vi "NSA Call Process.vi"(8 "error in (no error)":errorcluster caption="에러 입력(에러 없음)", 10 "NSA Call Process Param":T1, 11 "Instrument Manager 입력":refnum<class "Instrument Manager.lvclass">) -> (0 "error out":errorcluster caption="에러 출력", 3 "Instrument Manager 출력":refnum<class "Instrument Manager.lvclass">)   [LabVIEW 2023, in "Instrument Manager.lvclass"]
uses:
  Instrument Manager.lvclass
  Param Definition/NSA Call Process Param.ctl
  Module/ANRITSU Call Box/Type Definition/NR Modulation Type.ctl
  Instrument Manager.lvclass/Instrument Manager.ctl
  97ae3937-7c23-4982-aa73-e3704093bdd1.vi
  Module/ANRITSU Call Box/ANRITSU Call Box.lvlib
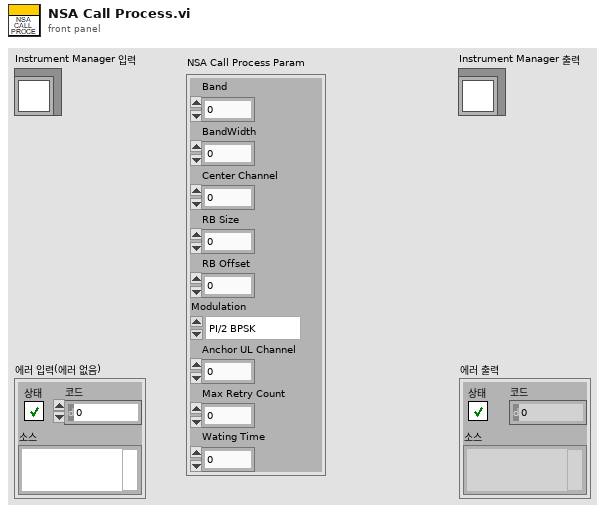
[diagram p1: front panel]
types:
  T1 = typedef "NSA Call Process Param.ctl" = cluster{"Band":u32, "BandWidth":u32, "Center Channel":u32, "RB Size":i32, "RB Offset":i32, "Modulation":T2, "Anchor UL Channel":i32, "Max Retry Count":i32, "Wating Time":i32}
  T2 = typedef "ANRITSU Call Box.lvlib/NR Modulation Type.ctl" = enum16{"PI/2 BPSK", "QPSK", "16QAM", "64QAM", "256QAM"}
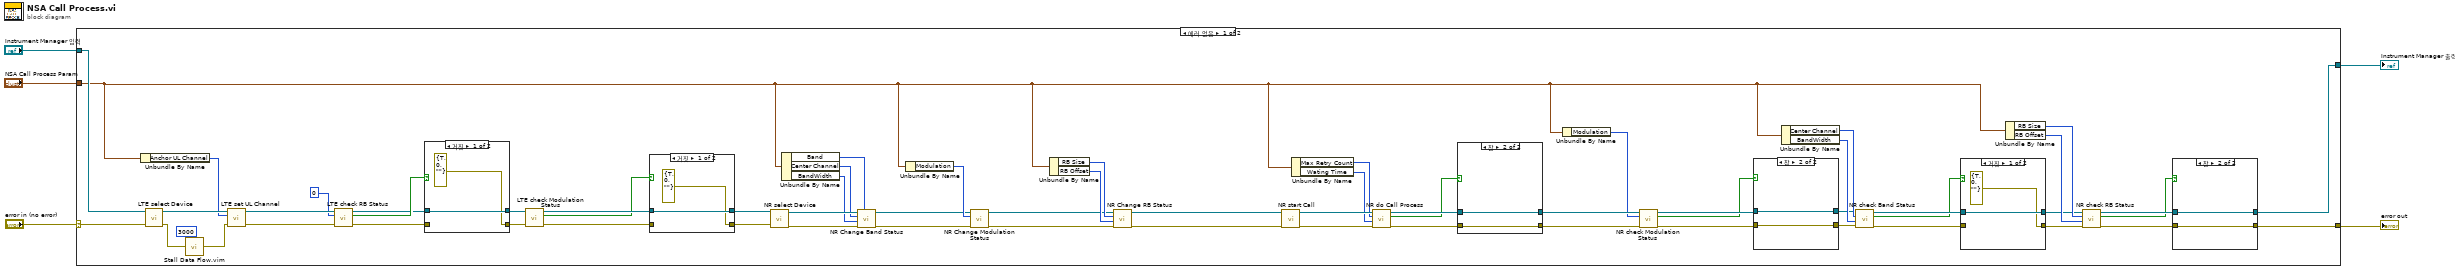
[diagram p0: block diagram]
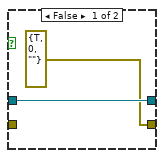
[diagram p2: hidden frame]
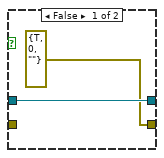
[diagram p4: hidden frame]
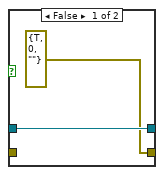
[diagram p5: hidden frame]
diagram:
  n1 = case shown="에러 없음" "error in (no error)" {
    selector: "error in (no error)" -> [w56 w95]
    tunnel: [w12 w95] -> w4
    tunnel: [w9 w94] -> w2
    tunnel: "Instrument Manager 입력" -> [w55 w94]
    tunnel: "NSA Call Process Param" -> [w21 _]
    frame No Error {
      n2 = Unbundle By Name(w21) -> ("Anchor UL Channel"=w58:i32)
      n3 = call "LTE select Device.vi"("error in (no error)"=w56, "Instrument Manager 입력"=w55) -> ("error out"=w8:errorcluster, "Instrument Manager 출력"=w61:refnum<class "Instrument Manager.lvclass">)  [unwired: 8 in]
      n4 = call "Stall Data Flow.vim"("value in"=w8, "milliseconds to wait"=u32 3000) -> ("value out"=w7:errorcluster)  [unwired: 1 out]
      n5 = call "LTE set UL Channel.vi"("error in (no error)"=w7, "UL Channel"=w58, "Instrument Manager 입력"=w61) -> ("error out"=w59:errorcluster, "Instrument Manager 출력"=w60:refnum<class "Instrument Manager.lvclass">)  [unwired: 7 in]
      n6 = call "LTE check RB Status.vi"("error in (no error)"=w59, "RB Offset"=0, "Instrument Manager 입력"=w60) -> ("error out"=w62:errorcluster, "불리언"=w64:bool, "Instrument Manager 출력"=w63:refnum<class "Instrument Manager.lvclass">)  [unwired: 6 in]
      n7 = case shown="거짓" w64 {
        tunnel: w63 -> [w91 w93]
        tunnel: [w91 w93] -> w66
        tunnel: [errorcluster {"status"=TRUE, "code"=0, "source"=""} ("error out") w92] -> w65
        tunnel: w62 -> [_ w92]
        frame False {
        }
        frame True {
        }
      }
      n8 = call "LTE check Modulation Status.vi"("error in (no error)"=w65, "Instrument Manager 입력"=w66) -> ("error out"=w68:errorcluster, "불리언"=w67:bool, "Instrument Manager 출력"=w69:refnum<class "Instrument Manager.lvclass">)  [unwired: 7 in]
      n9 = case shown="거짓" w67 {
        tunnel: w69 -> [w87 w89]
        tunnel: [w87 w89] -> w25
        tunnel: [errorcluster {"status"=TRUE, "code"=0, "source"=""} ("error out") w88] -> w26
        tunnel: w68 -> [_ w88]
        frame False {
        }
        frame True {
        }
      }
      n10 = call "NR select Device.vi"("error in (no error)"=w26, "Instrument Manager 입력"=w25) -> ("error out"=w53:errorcluster, "Instrument Manager 출력"=w54:refnum<class "Instrument Manager.lvclass">)  [unwired: 8 in]
      n11 = Unbundle By Name(w21) -> ("Band"=w31:u32, "Center Channel"=w30:u32, "BandWidth"=w29:u32)
      n12 = call "NR Change Band Status.vi"("Operation Band"=w31, "error in (no error)"=w53, "BW (MHz)"=w29, "Center Channel Number"=w30, "Instrument Manager 입력"=w54) -> ("error out"=w28:errorcluster, "Instrument Manager 출력"=w27:refnum<class "Instrument Manager.lvclass">)  [unwired: 5 in]
      n13 = Unbundle By Name(w21) -> ("Modulation"=w32:T2)
      n14 = call "NR Change Modulation Status.vi"("error in (no error)"=w28, "Modulation"=w32, "Instrument Manager 입력"=w27) -> ("error out"=w37:errorcluster, "Instrument Manager 출력"=w38:refnum<class "Instrument Manager.lvclass">)  [unwired: 7 in]
      n15 = Unbundle By Name(w21) -> ("RB Size"=w40:i32, "RB Offset"=w39:i32)
      n16 = call "NR Change RB Status.vi"("error in (no error)"=w37, "RB Offset"=w39, "RB Size"=w40, "Instrument Manager 입력"=w38) -> ("error out"=w49:errorcluster, "Instrument Manager 출력"=w51:refnum<class "Instrument Manager.lvclass">)  [unwired: 6 in]
      n17 = call "NR start Call.vi"("error in (no error)"=w49, "Instrument Manager 입력"=w51) -> ("error out"=w50:errorcluster, "Instrument Manager 출력"=w52:refnum<class "Instrument Manager.lvclass">)  [unwired: 8 in]
      n18 = Unbundle By Name(w21) -> ("Max Retry Count"=w45:i32, "Wating Time"=w44:i32)
      n19 = call "NR do Call Process.vi"("error in (no error)"=w50, "Waiting Time"=w44, "Max Retry Count"=w45, "Instrument Manager 입력"=w52) -> ("error out"=w43:errorcluster, "Connected?"=w41:bool, "Instrument Manager 출력"=w42:refnum<class "Instrument Manager.lvclass">)  [unwired: 5 in]
      n20 = case shown="참" w41 {
        tunnel: w42 -> [w83 w85]
        tunnel: [w83 w85] -> w47
        tunnel: [errorcluster {"status"=TRUE, "code"=0, "source"=""} ("error out") w84] -> w46
        tunnel: w43 -> [_ w84]
        frame False {
        }
        frame True {
        }
      }
      n21 = Unbundle By Name(w21) -> ("Modulation"=w33:T2)
      n22 = call "NR check Modulation Status.vi"("error in (no error)"=w46, "Modulation"=w33, "Instrument Manager 입력"=w47) -> ("error out"=w24:errorcluster, "Success?"=w22:bool, "Instrument Manager 출력"=w23:refnum<class "Instrument Manager.lvclass">)  [unwired: 6 in]
      n23 = case shown="참" w22 {
        tunnel: w23 -> [w79 w80]
        tunnel: [w79 w80] -> w20
        tunnel: [errorcluster {"status"=TRUE, "code"=0, "source"=""} ("error out") w81] -> w19
        tunnel: w24 -> [_ w81]
        frame False {
        }
        frame True {
        }
      }
      n24 = Unbundle By Name(w21) -> ("Center Channel"=w35:u32, "BandWidth"=w34:u32)
      n25 = call "NR check Band Status.vi"("error in (no error)"=w19, "BW (MHz)"=w34, "Center Channel Number"=w35, "Instrument Manager 입력"=w20) -> ("error out"=w18:errorcluster, "Success?"=w14:bool, "Instrument Manager 출력"=w17:refnum<class "Instrument Manager.lvclass">)  [unwired: 5 in]
      n26 = case shown="거짓" w14 {
        tunnel: w17 -> [w75 w77]
        tunnel: [w75 w77] -> w15
        tunnel: [errorcluster {"status"=TRUE, "code"=0, "source"=""} ("error out") w76] -> w16
        tunnel: w18 -> [_ w76]
        frame False {
        }
        frame True {
        }
      }
      n27 = Unbundle By Name(w21) -> ("RB Size"=w48:i32, "RB Offset"=w36:i32)
      n28 = call "NR check RB Status.vi"("error in (no error)"=w16, "RB Offset"=w36, "RB Size"=w48, "Instrument Manager 입력"=w15) -> ("error out"=w13:errorcluster, "Success?"=w10:bool, "Instrument Manager 출력"=w11:refnum<class "Instrument Manager.lvclass">)  [unwired: 5 in]
      n29 = case shown="참" w10 {
        tunnel: w11 -> [w71 w73]
        tunnel: [w71 w73] -> w9
        tunnel: [errorcluster {"status"=TRUE, "code"=0, "source"=""} ("error out") w72] -> w12
        tunnel: w13 -> [_ w72]
        frame False {
        }
        frame True {
        }
      }
    }
    frame Error {
    }
  }
  "error out" <- w4
  "Instrument Manager 출력" <- w2
